vi "Add Service.vi"(8 "error in (no error)":errorcluster, 10 "Service":refnum<class "Service.lvclass">, 11 "Server in":refnum<class "Server.lvclass">) -> (0 "error out":errorcluster, 3 "Server out":refnum<class "Server.lvclass">)   [LabVIEW 2020, in "HTTP Server.lvlib" / "Server.lvclass"]
doc: "Adds a Service to the server so it will be available during requests. Only a single instance of a service type can be registered with a server and if a type of service is registered a second time an error will be generated.\n\nCaution must be exercised when using shared resources in Services as this can lead to contention between parallel requests and significantly reduce request processing performance. Services are best implemented as stateless by-value classes. Services are not updated from request to request and are provided to each request with exactly the class private data values as it has when registered. The key idea is that services provide some functionality to every request and can be configured before being registered but since multiple requests can be processed simultaneously, services should ideally not cause contention between requests. Any changes made to a service in a request and written back to the Processing container will be not be shared among other requests. It is possible to use a service within a single request to store state for that request such as storing authentication information, retrieved database values, etc.\n\nIf a service needs to be configured for each individual request made, a pattern to follow can be registering an accompanying request handler with a low-ish priority (2000-10000) that has the sole resposibility of initializing the service for that request and updating it back into the processing container."
uses:
  Server.lvclass
  Service/Service.lvclass
  Server.lvclass/Server.ctl
  Values/Values.lvclass
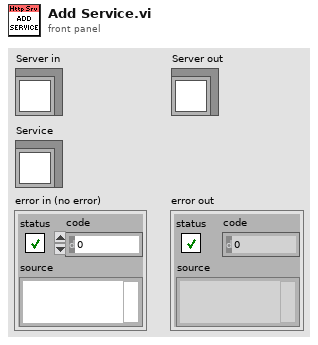
[diagram p1: front panel]
types:
  T1 = typedef "HTTP Server.lvlib/Server.lvclass/Ref Data.ctl" = cluster{"Connection Handler Map":T2, "Request Handler Map":T4, "Route Handler Map":T5, "Controller Handler Map":T6, "Controller Map":T7, "Response Handler Map":T8, "Complete Handler Map":T9, "Exception Handler Map":T10, "Connection Handler Index":u16, "Request Handler Index":u16, "Route Handler Index":u16, "Controller Handler Index":u16, "Controller Index":u16, "Response Handler Index":u16, "Complete Handler Index":u16, "Exception Handler Index":u16, "Values":refnum<class "Values.lvclass">, "Path":path, "Session Type":refnum<class "Session.lvclass">, "Session Cookie Name":string, "WebSocket Handler":refnum<class "WebSocket Handler.lvclass">, "WebSocket Handling":bool}
  T2 = typedef "HTTP Server.lvlib/Connection Handler Map.ctl" = map{T3, refnum<class "Connection Handler.lvclass">}
  T3 = typedef "HTTP Server.lvlib/Priority.ctl" = cluster{"Entity":u16, "Index":u16}
  T4 = typedef "HTTP Server.lvlib/Request Handler Map.ctl" = map{T3, refnum<class "Request Handler.lvclass">}
  T5 = typedef "HTTP Server.lvlib/Route Handler Map.ctl" = map{T3, refnum<class "Route Handler.lvclass">}
  T6 = typedef "HTTP Server.lvlib/Controller Handler Map.ctl" = map{T3, refnum<class "Controller Handler.lvclass">}
  T7 = typedef "HTTP Server.lvlib/Controller Map.ctl" = map{T3, refnum<class "Controller.lvclass">}
  T8 = typedef "HTTP Server.lvlib/Response Handler Map.ctl" = map{T3, refnum<class "Response Handler.lvclass">}
  T9 = typedef "HTTP Server.lvlib/Complete Handler Map.ctl" = map{T3, refnum<class "Complete Handler.lvclass">}
  T10 = typedef "HTTP Server.lvlib/Exception Handler Map.ctl" = map{T3, refnum<class "Exception Handler.lvclass">}
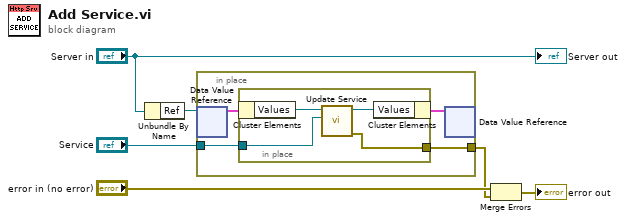
[diagram p0: block diagram]
diagram:
  n1 = Unbundle By Name("Server in") -> ("Ref"=w5:refnum<data-value>)
  n2 = in-place {
    in-place-border: "Service" -> [w8]
    in-place-border: [w7] -> w1
    n3 = in-place-dvr #1(w5) -> (w10:T1)  [unwired: 1 out]
    n4 = in-place {
      in-place-border: w8 -> [w11]
      in-place-border: [w12] -> w7
      n5 = in-place-cluster #2(w10) -> ("Values"=w14:refnum<class "Values.lvclass">)
      n6 = call "Update Service.vi"("Service"=w11, "Values in"=w14) -> ("error out"=w12:errorcluster, "Values out"=w13:refnum<class "Values.lvclass">)  [unwired: 8 in]
      n7 = in-place-cluster #2("Values"=w13) -> (w9:T1)
    }
    n8 = in-place-dvr #1(w9) -> ()  [unwired: 2 out]
  }
  n9 = Merge Errors("error in (no error)", w1) -> (→"error out":errorcluster)
  "Server out" <- "Server in"
